vi "CIVI Read Session Example.vi"() -> ()   [LabVIEW 2026]
panel:
  out "S Meter (raw)":i32
  out "Mode":string
  out "error out":errorcluster
  out "Frequency (Hz)":i32
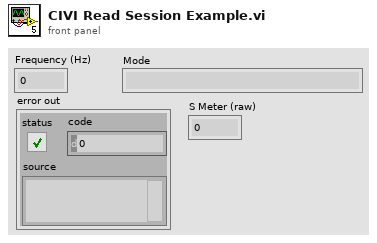
[diagram p1: front panel]
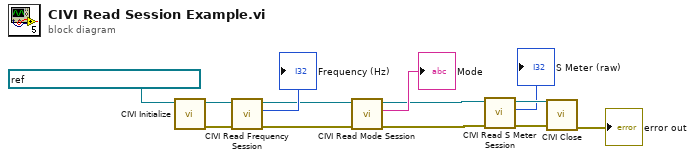
[diagram p0: block diagram]
diagram:
  n1 = call "CIVI Initialize.vi"("VISA Resource Name"=refnum<visa-resource-name> "TCPIP0::127.0.0.1::5025::SOCKET") -> ("error out"=w13:errorcluster, "VISA Session out"=w12:refnum<visa-resource-name>)  [unwired: 9 in]
  n2 = call "CIVI Read Frequency Session.vi"("error in"=w13, "VISA Session in"=w12) -> ("error out"=w7:errorcluster, "Frequency (Hz)"=→"Frequency (Hz)":i32, "VISA Session out"=w8:refnum<visa-resource-name>)  [unwired: 7 in]
  n3 = call "CIVI Read Mode Session.vi"("error in"=w7, "VISA Session in"=w8) -> ("error out"=w2:errorcluster, "Mode"=→"Mode":string, "VISA Session out"=w3:refnum<visa-resource-name>)  [unwired: 7 in]
  n4 = call "CIVI Read S Meter Session.vi"("error in"=w2, "VISA Session in"=w3) -> ("error out"=w5:errorcluster, "S Meter (raw)"=→"S Meter (raw)":i32, "VISA Session out"=w4:refnum<visa-resource-name>)  [unwired: 7 in]
  n5 = call "CIVI Close.vi"("error in"=w5, "VISA Session in"=w4) -> ("error out"=→"error out":errorcluster)  [unwired: 9 in]
